vi "AssertValueByFocusName.vi"(0 "VI Reference In":refnum<vi>, 1 "Test Label":string, 2 "delimiter (>>)":string=">>", 3 "Assert Only? (F)":bool, 5 "Control Path":string, 7 "Item Name":string, 11 "Error In":errorcluster, 12 "Assert Interval(10 ms)":u32=10, 13 "Timeout(5 sec)":dbl=5.0) -> (4 "VI Reference Out":refnum<vi>, 6 "Asserted Value":string, 15 "Error Out":errorcluster)   [LabVIEW 2016, in "Drona.lvlib" / "AssertControlValue.lvlib" / "AssertListbox.lvlib"]
doc: "Asserts if the focus item name on listbox controls is equal.\n\nThe input control name is given as a string , incase of path, use delimiters inbetween the path.\nThis VI gets the value of the control, untill the value is equal to the input value."
uses:
  AssertListbox.lvlib
  Get/GetControlRef/GetControlRefByPath.vi
  <vilib>/Utility/error.llb/Error Cluster From Error Code.vi
  <vilib>/addons/_JKI Toolkits/Caraya/classes/Assert/Assert Equal Value_Variant.vi
  <vilib>/ErrorRing/Error Ring.xnode
  <vilib>/addons/_JKI Toolkits/Caraya/classes/Assert/Assert.lvclass
  Get/GetControlRef/GetControlRef.lvlib
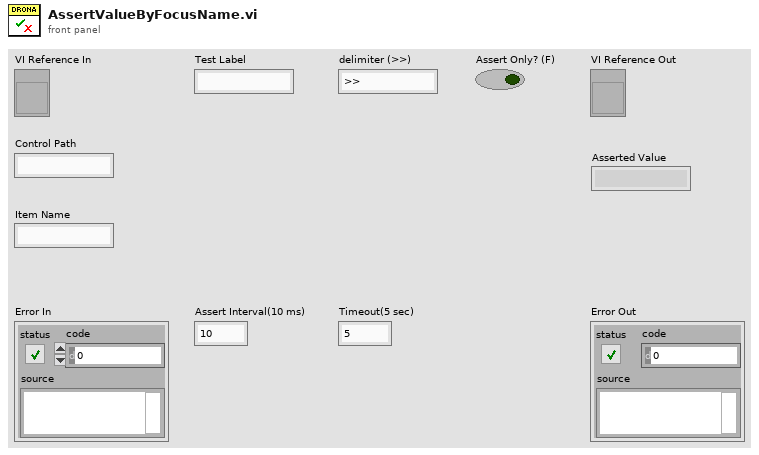
[diagram p1: front panel]
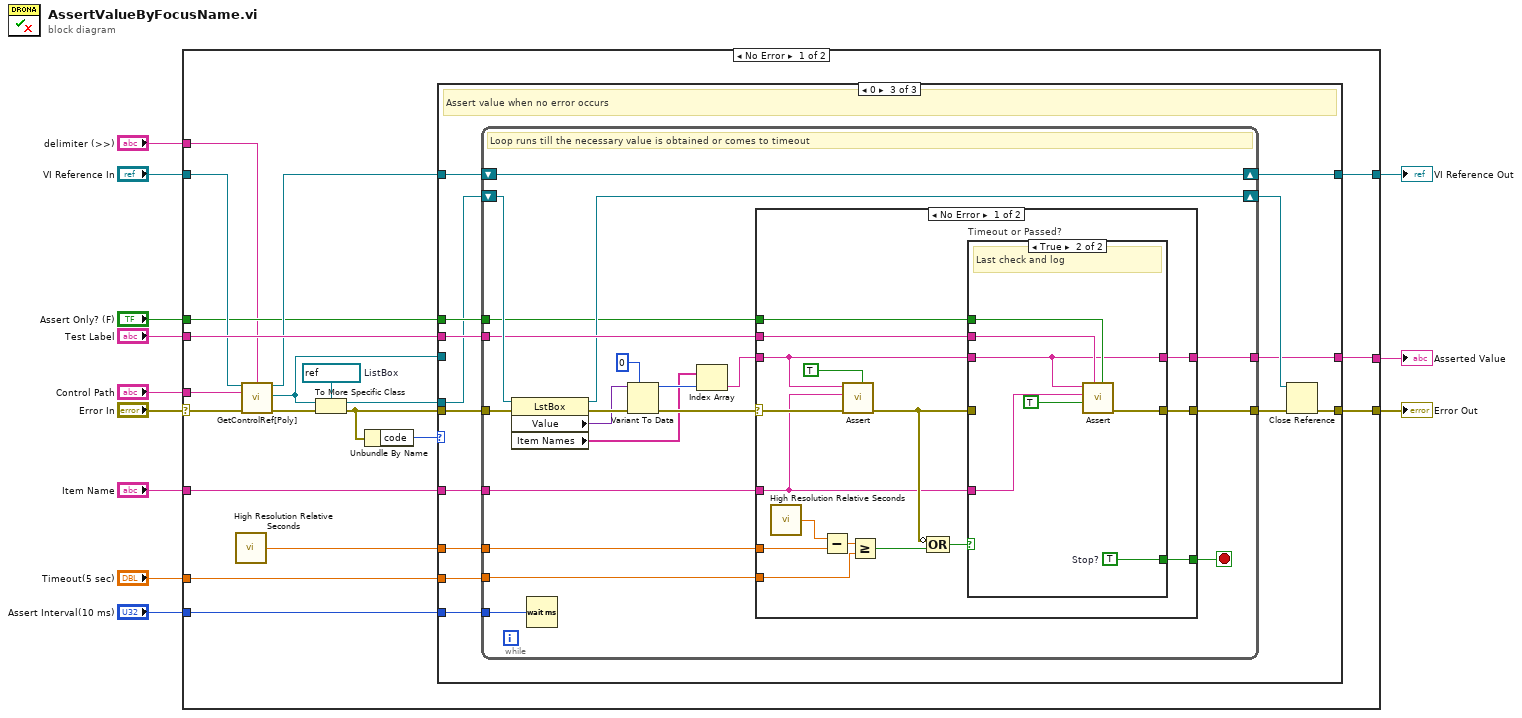
[diagram p0: block diagram]
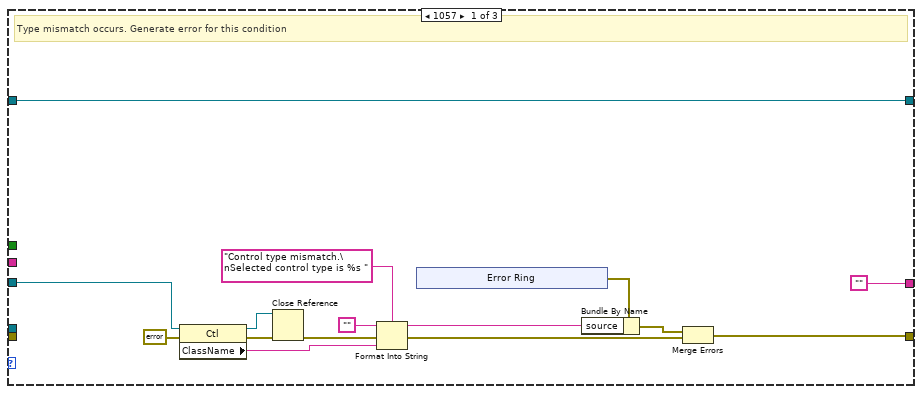
[diagram p2: hidden frame]
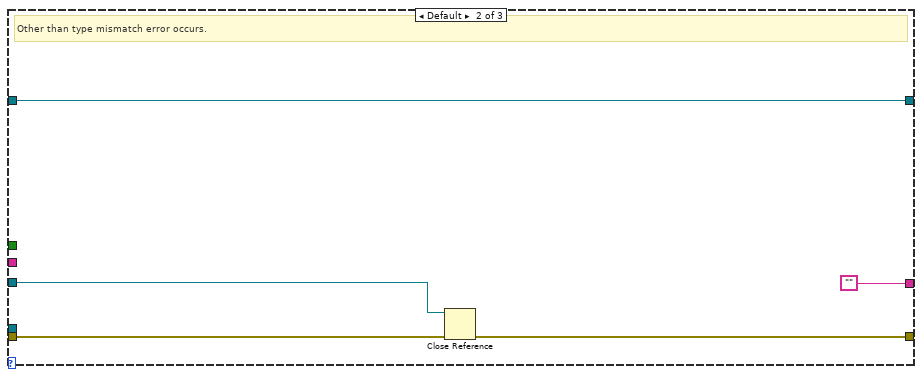
[diagram p3: hidden frame]
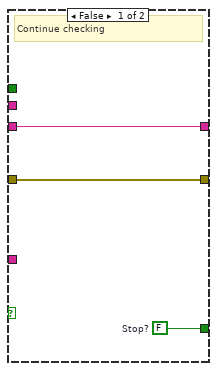
[diagram p4: hidden frame]
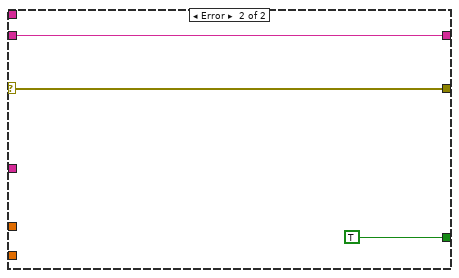
[diagram p5: hidden frame]
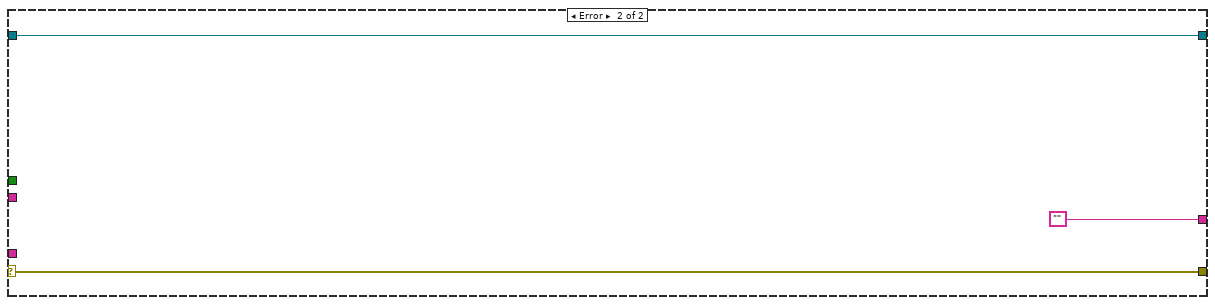
[diagram p6: hidden frame]
diagram:
  n1 = case shown="No Error" "Error In" {
    selector: "Error In" -> [w27 w123]
    tunnel: "Timeout(5 sec)" -> [w32 _]
    tunnel: [w31 w122] -> w11
    tunnel: "Item Name" -> [w30 _]
    tunnel: [w22 w123] -> w10
    tunnel: "Assert Interval(10 ms)" -> [w29 _]
    tunnel: "Test Label" -> [w28 _]
    tunnel: "VI Reference In" -> [w26 w122]
    tunnel: "Control Path" -> [w13 _]
    tunnel: "delimiter (>>)" -> [w14 _]
    tunnel: "Assert Only? (F)" -> [w21 _]
    tunnel: [w20 ""] -> w1
    frame No Error {
      w19 = refnum<vi> refnum  # ListBox
      n2 = call <vilib>:"High Resolution Relative Seconds.vi"() -> ("relative seconds"=w25:dbl)
      n3 = call-poly "GetControlRef[Poly].vi"("VI Reference In"=w26, "delimiter (>>)"=w14, "Control Path"=w13, "error In"=w27) -> ("VI Reference Out"=w23:refnum<vi>, "Ctl Refnum"=w15:refnum<vi>, "error out"=w24:errorcluster)  [unwired: 9 in]
      n4 = To More Specific Class(target class=w19, reference=w15, error in=w24) -> (specific class reference=w18:refnum<vi>, error out=w17:errorcluster)
      n5 = Unbundle By Name(w17) -> ("code"=w16:i32)
      n6 = case shown="0" w16 {
        tunnel: w32 -> [_ _ w71]
        tunnel: [w47 w57 w70] -> w31
        tunnel: w30 -> [_ _ w69]
        tunnel: w29 -> [_ _ w67]
        tunnel: w28 -> [_ _ w66]
        tunnel: w25 -> [_ _ w65]
        tunnel: w23 -> [w47 w57 w64]
        tunnel: [w34 w54 w63] -> w22
        tunnel: w21 -> [_ _ w61]
        tunnel: ["" "" w60] -> w20
        tunnel: w17 -> [_ w56 w59]
        tunnel: w18 -> [_ _ w58]
        tunnel: w15 -> [w33 w53 _]
        frame 1057 {
          # "Type mismatch occurs. Generate error for this condition"
          n7 = property class="Ctl"(reference=w33, error in=errorcluster {"status"=FALSE, "code"=0, "source"=""} ("error out")) -> (reference out=w35:refnum<vi>, error out=w45:errorcluster, "ClassName"=w42:string)
          n8 = Close Reference(reference=w35, error in (no error)=w45) -> (error out=w36:errorcluster)
          n9 = Format Into String(format string="Control type mismatch.\nSelected control type is %s ", initial string="", error in=w36, w42) -> (resulting string=w39:string, error out=w37:errorcluster)
          n10 = xnode "Error Ring"() -> ("error out"=w40:errorcluster)
          n11 = Bundle By Name(cluster=w40, "source"=w39) -> (w38:errorcluster)
          n12 = Merge Errors(w38, w37) -> (w34:errorcluster)
        }
        frame Default {
          # "Other than type mismatch error occurs."
          n13 = Close Reference(reference=w53, error in (no error)=w56) -> (error out=w54:errorcluster)
        }
        frame 0 {
          # "Assert value when no error occurs"
          n14 = while {
            tunnel: w69 -> [w78]
            tunnel: w71 -> [w90]
            tunnel: w65 -> [w91]
            tunnel: w59 -> [w85]
            tunnel: [w88] -> w68
            tunnel: w67 -> [w86]
            tunnel: w66 -> [w82]
            shift-right: [w83] -> w70
            shift-left: w64 -> [w83]
            shift-right: [w81] -> w62
            shift-left: w58 -> [w84]
            tunnel: w61 -> [w80]
            tunnel: [w79] -> w60
            stop <- w89 stop-if-true
            # "Loop runs till the necessary value is obtained or comes to timeout"
            n15 = property on="Property Node" class="LstBox"(reference=w84, error in=w85) -> (reference out=w81:refnum<vi>, error out=w87:errorcluster, "Value"=w76:variant, "Item Names"=w72:string[])
            n16 = Wait (ms)(milliseconds to wait=w86) -> ()  [unwired: 1 out]
            n17 = Variant To Data(error in=w87, type=0, Variant=w76) -> (data=w74:i32, error out=w77:errorcluster)
            n18 = Index Array(array=w72, index=w74) -> (element=w73:string)
            n19 = case shown="No Error" w77 {
              selector: w77 -> [w103 w120]
              tunnel: w91 -> [w107 _]
              tunnel: w90 -> [w104 _]
              tunnel: [w94 TRUE] -> w89
              tunnel: [w95 w120] -> w88
              tunnel: w78 -> [w96 _]
              tunnel: w73 -> [w97 w118]
              tunnel: w82 -> [w102 _]
              tunnel: w80 -> [w93 _]
              tunnel: [w92 w118] -> w79
              frame No Error {
                n20 = call <vilib>:"High Resolution Relative Seconds.vi"() -> ("relative seconds"=w106:dbl)
                n21 = Subtract(x=w106, y=w107) -> (x-y=w105:dbl)
                n22 = call-poly <vilib>:"Assert.vi"("Assert Only? (F)"=TRUE, "error in (no error)"=w103, "Y"=w96, "X"=w97) -> ("error out"=w100:errorcluster)  [unwired: 6 in, 1 out]
                n23 = Greater Or Equal?(x=w105, y=w104) -> (x >= y?=w101:bool)
                n24 = Compound Arithmetic op=OR(invert w100, w101) -> (w99:bool)
                n25 = case "Timeout or Passed?" shown="True" w99 {
                  tunnel: w100 -> [w110 _]
                  tunnel: w96 -> [_ w113]
                  tunnel: w97 -> [w108 w112]
                  tunnel: w102 -> [_ w117]
                  tunnel: [w110 w116] -> w95
                  tunnel: [w109 w115] -> w94
                  tunnel: w93 -> [_ w114]
                  tunnel: [w108 w112] -> w92
                  frame False {
                    w109 = FALSE  # Stop?
                    # "Continue checking"
                  }
                  frame True {
                    w115 = TRUE  # Stop?
                    # "Last check and log"
                    n26 = call-poly <vilib>:"Assert.vi"("Assert Only? (F)"=w114, "Label"=w117, "Register with caller test (F)"=TRUE, "Y"=w113, "X"=w112) -> ("error out"=w116:errorcluster)  [unwired: 5 in, 1 out]
                  }
                }
              }
              frame Error {
              }
            }
          }
          n27 = Close Reference(reference=w62, error in (no error)=w68) -> (error out=w63:errorcluster)
        }
      }
    }
    frame Error {
    }
  }
  "Error Out" <- w10
  "VI Reference Out" <- w11
  "Asserted Value" <- w1
